vi "Glyphs_Blit.vi"(0 "Picture":u8[][](array[numeric]), 5 "Sprites":cluster{"Pix":u8[][], "Mask":u8[][]}[](array[cluster]), 7 "Text":string, 9 "Position":cluster{"X":i32, "Y":i32}, 11 "error in":errorcluster) -> (4 "Picture out":u8[][](array[numeric]), 15 "error out":errorcluster)   [LabVIEW 2020, in "GH_Render.lvlib"]
doc: "Writes Text with the glyph sprites (characters \"ABCDEFGHIJKLMNOPQRSTUVWXYZ0123456789 .:-!=\", 24 px apart) from Position (top left). Unknown characters and spaces stay empty."
uses:
  GH_Render.lvlib
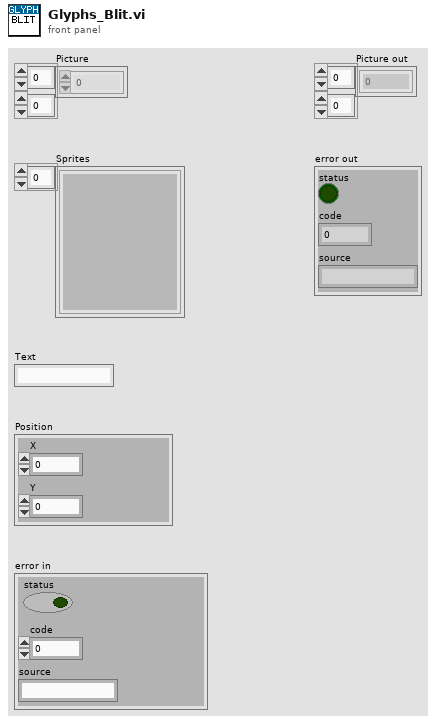
[diagram p1: front panel]
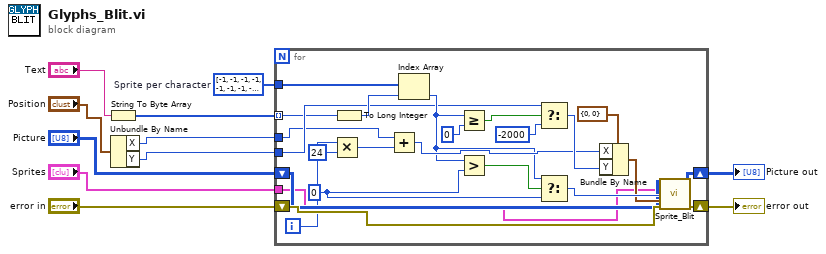
[diagram p0: block diagram]
diagram:
  w8 = i32[] [-1, -1, -1, -1, -1, -1, -1, -1, -1, -1, -1, -1, -1, -1, -1, -1, -1, -1, -1, -1, -1, -1, -1, -1, -1, -1, -1, -1, -1, -1, -1, -1, -1, 99, -1, -1, -1, -1, -1, -1, -1, -1, -1, -1, -1, 98, 96, -1, 85, 86, 87, 88, 89, 90, 91, 92, 93, 94, 97, -1, -1, 100, -1, -1, -1, 59, 60, 61, 62, 63, 64, 65, 66, 67, 68, 69, 70, 71, 72, 73, 74, 75, 76, 77, 78, 79, 80, 81, 82, 83, 84, -1, -1, -1, -1, -1, -1, -1, -1, -1, -1, -1, -1, -1, -1, -1, -1, -1, -1, -1, -1, -1, -1, -1, -1, -1, -1, -1, -1, -1, -1, -1, -1, -1, -1, -1, -1, -1, -1, -1, -1, -1, -1, -1, -1, -1, -1, -1, -1, -1, -1, -1, -1, -1, -1, -1, -1, -1, -1, -1, -1, -1, -1, -1, -1, -1, -1, -1, -1, -1, -1, -1, -1, -1, -1, -1, -1, -1, -1, -1, -1, -1, -1, -1, -1, -1, -1, -1, -1, -1, -1, -1, -1, -1, -1, -1, -1, -1, -1, -1, -1, -1, -1, -1, -1, -1, -1, -1, -1, -1, -1, -1, -1, -1, -1, -1, -1, -1, -1, -1, -1, -1, -1, -1, -1, -1, -1, -1, -1, -1, -1, -1, -1, -1, -1, -1, -1, -1, -1, -1, -1, -1, -1, -1, -1, -1, -1, -1, -1, -1, -1, -1, -1, -1, -1, -1, -1, -1, -1, -1, -1, -1, -1, -1, -1, -1]  # Sprite per character
  n1 = String To Byte Array(string="Text") -> (unsigned byte array=w9:u8[])
  n2 = Unbundle By Name("Position") -> ("X"=w6:i32, "Y"=w7:i32)
  n3 = for {
    tunnel: w8 -> [w14]
    tunnel: "Sprites" -> [w15]
    shift-right: [w19] -> w10
    shift-left: "Picture" -> [w18]
    shift-right: [w21] -> w11
    shift-left: "error in" -> [w20]
    tunnel: w9 -> [w13] mode=indexing
    tunnel: w6 -> [w16]
    tunnel: w7 -> [w17]
    i -> [w12]
    w33 = 0
    n4 = Multiply(x=w12, y=24) -> (x*y=w28:i32)
    n5 = To Long Integer(number=w13) -> (32bit integer=w22:i32)
    n6 = Add(x=w16, y=w28) -> (x+y=w29:i32)
    n7 = Index Array(array=w14, index=w22) -> (element=w23:i32)
    n8 = Greater Or Equal?(x=w23, y=0) -> (x >= y?=w25:bool)
    n9 = Greater?(x=w23, y=w33) -> (0:w34:bool)
    n10 = Select(t=w17, s=w25, f=-2000) -> (s? t:f=w31:i32)
    n11 = Select(t=w23, s=w34, f=w33) -> (s? t:f=w35:i32)
    n12 = Bundle By Name(cluster=cluster{"X":i32, "Y":i32} {"X"=0, "Y"=0}, "X"=w29, "Y"=w31) -> (w32:cluster{"X":i32, "Y":i32})
    n13 = call "Sprite_Blit.vi"("Picture"=w18, "Sprites"=w15, "Index"=w35, "Position"=w32, "error in"=w20) -> ("Picture out"=w19:u8[][], "error out"=w21:errorcluster)  [unwired: 9 in]
  }
  "Picture out" <- w10
  "error out" <- w11
